vi "lvmcp_setcasenames.vi"() -> ()   [LabVIEW 2015]
panel:
  out "error out":errorcluster
  in  "names":string[](array[string])
  in  "reference":refnum<vi>
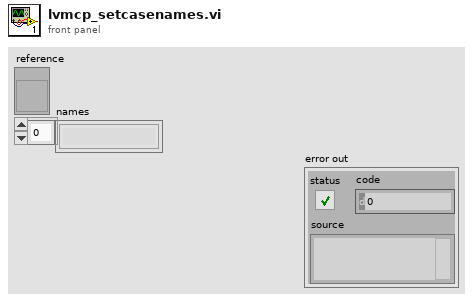
[diagram p1: front panel]
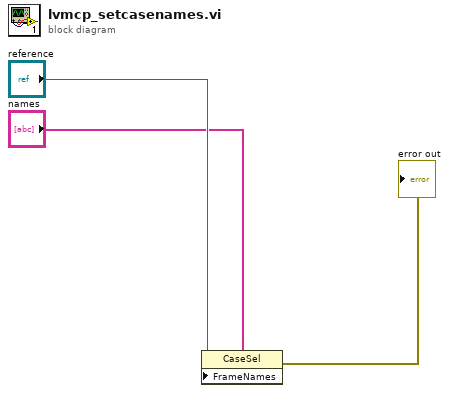
[diagram p0: block diagram]
diagram:
  n1 = property class="CaseSel"(reference="reference", "FrameNames"="names") -> (error out=→"error out":errorcluster)  [unwired: 1 in, 1 out]
